vi "Panel.vi"(11 "SubClone in":refnum<class "SubClone.lvclass">) -> ()   [LabVIEW 2020, in "SubPanels.lvlib" / "SubClone.lvclass"]
uses:
  SubClone.lvclass
  OOPanel/Panel/Panel.lvclass
  OOPanel/OOPanel.lvlib
panel:
  out "Iterations":i32
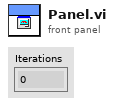
[diagram p1: front panel]
types:
  T1 = enum32{"Invalid", "Standard", "Closed", "Hidden", "Minimized", "Maximized"}
  T2 = typedef "OOPanel.lvlib/Visibility State.ctl" = enum16{"Idle", "Closed", "Hidden", "Visible", "Subpanel", "Hidden Subpanel"}
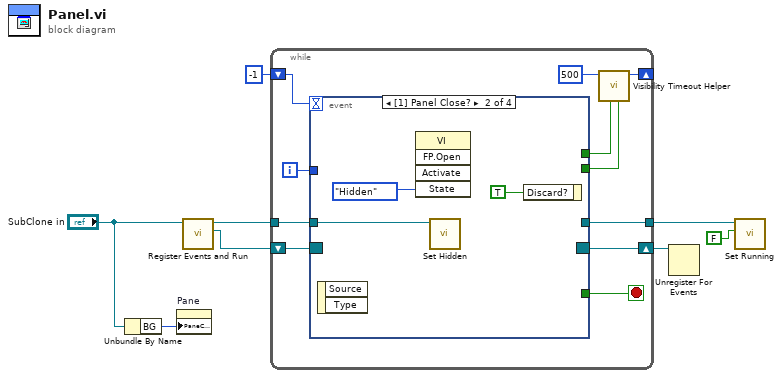
[diagram p0: block diagram]
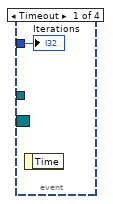
[diagram p2: hidden frame]
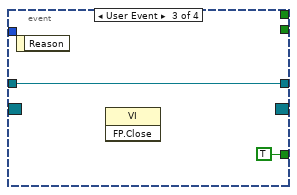
[diagram p3: hidden frame]
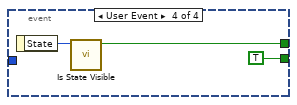
[diagram p4: hidden frame]
diagram:
  n1 = Unbundle By Name("SubClone in") -> ("BG"=w8:u32)
  n2 = property on="Pane" class="Pane"("PaneColor"=w8) -> ()  [unwired: 2 in, 2 out]
  n3 = call "Register Events and Run.vi"("Panel in"="SubClone in") -> ("Panel Event Reg"=w6:refnum<event-registration>, "Panel out"=w7:refnum<class "SubClone.lvclass">)  [unwired: 8 in, 1 out]
  n4 = while {
    tunnel: w7 -> [w10]
    shift-right: [w18] -> w2
    shift-left: w6 -> [w19]
    shift-right: [w16] -> _
    shift-left: -1 -> [w15]
    tunnel: [w9] -> w4
    i -> [w12]
    stop <- w11 stop-if-true
    n5 = event shown="[1] Panel Close?" {
      selector: w19 -> [_ _ _ _]
      dyn-events: [_ _ _ _] -> w18
      timeout: w15 -> [_ _ _ _]
      tunnel: [_ _ _ w27] -> w14
      tunnel: [_ _ _ TRUE] -> w13
      tunnel: w12 -> [w20 _ _ _]
      tunnel: [_ _ TRUE _] -> w11
      tunnel: w10 -> [_ w21 w24 _]
      tunnel: [_ _ w24 _] -> w9
      event Timeout {
        n6 = event-data() -> ()  [unwired: 1 in, 1 out]
        "Iterations" <- w20
      }
      event Panel Close? {
        n7 = event-data() -> ()  [unwired: 1 in, 2 out]
        n8 = invoke class="VI" method="FP.Open"("State"=T1."Hidden") -> ()  [unwired: 4 in, 5 out]
        n9 = call "Set Hidden.vi"("Panel in"=w21) -> ()  [unwired: 9 in, 2 out]
        n10 = event-data("Discard?"=TRUE) -> ()  [unwired: 1 in, 1 out]
      }
      event User Event {
        n11 = event-data() -> ()  [unwired: 1 in, 1 out]
        n12 = invoke class="VI" method="FP.Close"() -> ()  [unwired: 3 in, 3 out]
      }
      event User Event {
        n13 = event-data() -> ("State"=w28:T2)  [unwired: 1 in]
        n14 = call "Is State Visible.vi"("Visibility"=w28) -> ("Visible"=w27:bool)  [unwired: 10 in]
      }
    }
    n15 = call "Visibility Timeout Helper.vi"("Update?"=w13, "Use Timeout?"=w14, "Visible Timeout mS"=500) -> ("Timeout"=w16:i32)  [unwired: 8 in]
  }
  n16 = Unregister For Events(event registration refnum=w2) -> ()  [unwired: 1 in, 1 out]
  n17 = call "Set Running.vi"("Running"=FALSE, "Panel in"=w4) -> ()  [unwired: 8 in, 2 out]
